vi "Test WS Internet Echo.vi"(8 "error in (no error)":errorcluster, 11 "TestCase in":refnum<class "Test WebSocket Client.lvclass">) -> (0 "error out":errorcluster, 3 "TestCase out":refnum<class "Test WebSocket Client.lvclass">)   [LabVIEW 2013, in "Test WebSocket Client.lvclass"]
uses:
  Test WebSocket Client.lvclass
  WebSockets/WebSocket Client/WebSocket Client.lvclass
  WebSockets/WebSocket/WebSocket.lvclass/WebSocket.ctl
  <vilib>/addons/_JKI Toolkits/VI Tester/TestCase.llb/TestCase.lvclass
  WebSockets/WebSocket/WebSocket.lvclass
panel:
  out "Server Headers Out":variant
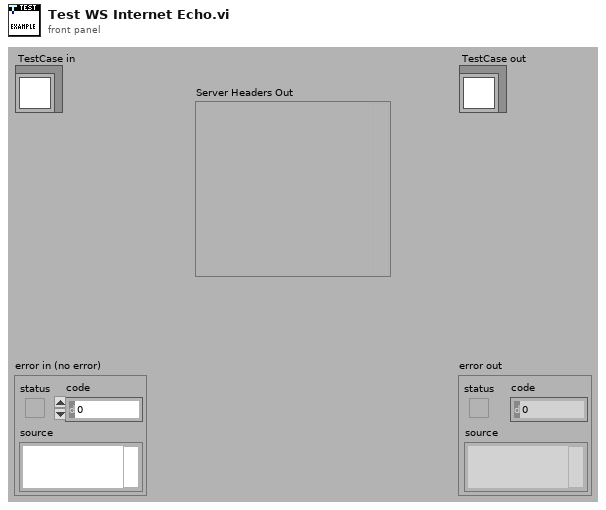
[diagram p1: front panel]
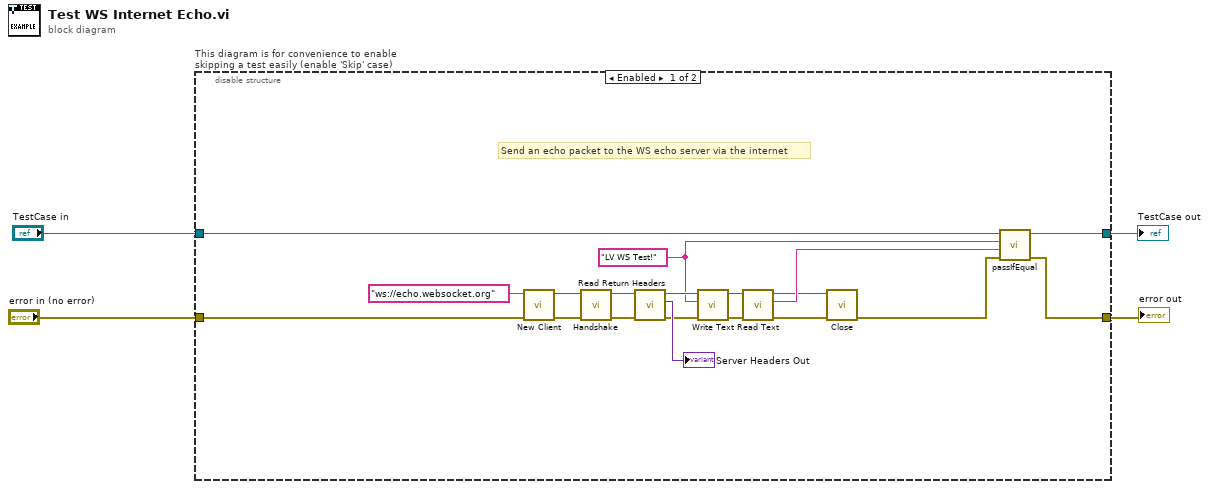
[diagram p0: block diagram]
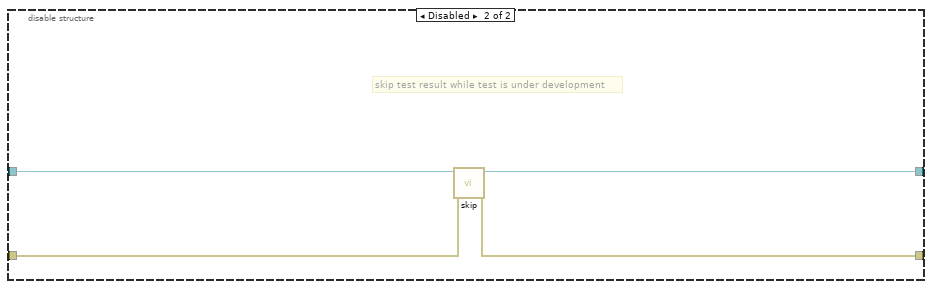
[diagram p2: hidden frame]
diagram:
  n1 = disable-structure "This diagram is for convenience to enable skipping a test easily (enable 'Skip' case)" shown="Enabled" {
    disable-tunnel: "TestCase in" -> [w23 w27]
    disable-tunnel: [w22 w25] -> w1
    disable-tunnel: [w21 w26] -> w3
    disable-tunnel: "error in (no error)" -> [w8 w24]
    frame Enabled {
      w14 = "LV WS Test!"
      # "Send an echo packet to the WS echo server via the internet"
      n2 = call "New Client.vi"("error in (no error)"=w8, "WebSocket URL"="ws://echo.websocket.org" ("address")) -> ("error out"=w7:errorcluster, "WebSocket Client out"=w6:refnum<class "WebSocket Client.lvclass">)  [unwired: 8 in]
      n3 = call-dynamic "Handshake.vi"("error in (no error)"=w7, "WebSocket Client in"=w6) -> ("error out"=w20:errorcluster, "WebSocket Client out"=w12:refnum<class "WebSocket Client.lvclass">)  [unwired: 8 in]
      n4 = call "Read Return Headers.vi"("error in (no error)"=w20, "WebSocket in"=w12) -> ("error out"=w18:errorcluster, "Return Headers"=→"Server Headers Out":variant, "WebSocket out"=w15:refnum<class "WebSocket Client.lvclass">)  [unwired: 7 in]
      n5 = call-dynamic "Write Text.vi"("error in (no error)"=w18, "String Data"=w14, "WebSocket in"=w15) -> ("error out"=w17:errorcluster, "WebSocket out"=w16:refnum<class "WebSocket Client.lvclass">)  [unwired: 7 in]
      n6 = call-dynamic "Read Text.vi"("error in (no error)"=w17, "WebSocket in"=w16) -> ("error out"=w11:errorcluster, "Data"=w13:string, "WebSocket out"=w10:refnum<class "WebSocket Client.lvclass">)  [unwired: 7 in]
      n7 = call-dynamic "Close.vi"("error in (no error)"=w11, "WebSocket in"=w10) -> ("error out"=w9:errorcluster)  [unwired: 9 in]
      n8 = call-dynamic "passIfEqual.vi"("error in (no error)"=w9, "y"=w13, "x"=w14, "TestCase in"=w23) -> ("error out"=w21:errorcluster, "TestCase out"=w22:refnum<class "Test WebSocket Client.lvclass">)  [unwired: 6 in]
    }
    frame Disabled {
      # "skip test result while test is under development"
      n9 = call <vilib>:"skip.vi"("error in (no error)"=w24, "TestCase in"=w27) -> ("error out"=w26:errorcluster, "TestCase out"=w25:refnum<class "Test WebSocket Client.lvclass">)  [unwired: 8 in]
    }
  }
  "error out" <- w3
  "TestCase out" <- w1
